vi "externalSetParam.vi"(0 "reference":refnum<class "ClassRelationshipEdge.lvclass">, 1 "arrowHead":T2, 2 "string":string, 3 "node":refnum<class "AbstractNode.lvclass">, 4 "bentStyle":T3, 5 "error in (no error)":errorcluster, 6 "setParam":T4, 7 "ConnectionOffset":cluster{"x":i32, "y":i32}, 9 "lineStyle":T1 caption="stroke") -> (14 "reference out":refnum<class "ClassRelationshipEdge.lvclass">, 19 "error out":errorcluster)   [LabVIEW 2020, in "ClassRelationshipEdge.lvclass"]
doc: "Sets externaly parameters on object"
uses:
  <resource>/Framework/Providers/Open_GDS/UML/ClassRelationshipEdge_class/ClassRelationshipEdge.lvclass
  C:/Program Files (x86)/National Instruments/LabVIEW 2020/resource/Framework/Providers/Open_GDS/UML/SegmentedLineEdge_class/SegmentedLineEdge.lvclass
  C:/Program Files (x86)/National Instruments/LabVIEW 2020/resource/Framework/Providers/Open_GDS/UML/AbstractEdge_class/AbstractEdge.lvclass
  <resource>/Framework/Providers/Open_GDS/UML/ClassRelationshipEdge_class/ExternaSetParamType.ctl
  <resource>/Framework/Providers/Open_GDS/UML/AbstractNode_class/AbstractNode.lvclass
  <resource>/Framework/Providers/Open_GDS/UML/BentStyle_class/BentStyleType.ctl
  <resource>/Framework/Providers/Open_GDS/UML/ArrowHead_class/ArrowHeadType.ctl
  <resource>/Framework/Providers/Open_GDS/UML/LineStyle_class/LineStyleType.ctl
  <resource>/Framework/Providers/Open_GDS/UML/ArrowHead_class/ArrowHead.lvclass
  <resource>/Framework/Providers/Open_GDS/UML/BentStyle_class/BentStyle.lvclass
  <resource>/Framework/Providers/Open_GDS/UML/SegmentedLineEdge_class/SegmentedLineEdge.lvclass
  <resource>/Framework/Providers/Open_GDS/UML/AbstractEdge_class/AbstractEdge.lvclass
  <resource>/Framework/Providers/Open_GDS/UML/LineStyle_class/LineStyle.lvclass
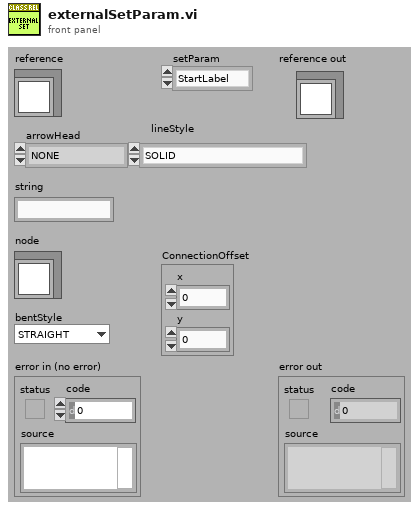
[diagram p1: front panel]
types:
  T1 = typedef "LineStyle.lvclass/LineStyleType.ctl" = enum16{"SOLID", "DOTTED"}
  T2 = typedef "ArrowHead.lvclass/ArrowHeadType.ctl" = enum16{"NONE", "TRIANGLE", "BLACK_TRIANGLE", "V", "HALF_V", "DIAMOND", "BLACK_DIAMOND"}
  T3 = typedef "BentStyle.lvclass/BentStyleType.ctl" = enum16{"STRAIGHT", "HV", "VH", "HVH", "VHV", "ARC"}
  T4 = typedef "ClassRelationshipEdge.lvclass/ExternaSetParamType.ctl" = enum16{"StartLabel", "MidLabel", "EndLabel", "StartNode", "EndNode", "BendType", "StartArrow", "EndArrow", "StartOffset", "EndOffset", "LineStyle"}
  T5 = typedef "ClassRelationshipEdge.lvclass/ObjectAttributes.ctl" = cluster{"bentStyleRef":refnum<class "BentStyle.lvclass">, "startConnectionOffset":cluster{"x":i32, "y":i32}, "endConnectionOffset":cluster{"x":i32, "y":i32}, "MidLineOffset":cluster{"x":i32, "y":i32}, "DepClass":T6}
  T6 = typedef "ReversedEngineering_ViDependencyDetailsType.ctl" = cluster{"ThisVIs/Ctls":path[], "Dependent_VIs/Ctls":path[]}
  T7 = typedef "SegmentedLineEdge.lvclass/ObjectAttributes.ctl" = cluster{"lineStyle":refnum<class "LineStyle.lvclass">, "startArrowHead":refnum<class "ArrowHead.lvclass">, "endArrowHead":refnum<class "ArrowHead.lvclass">, "startLabel":string, "midLabel":string, "endLabel":string, "MidLabelOffset":T8, "SplitWire":bool}
  T8 = typedef "Point Point2D.ctl" = cluster{"x":dbl, "y":dbl}
  T9 = typedef "AbstractEdge.lvclass/ObjectAttributes.ctl" = cluster{"start":refnum<class "AbstractNode.lvclass">, "end":refnum<class "AbstractNode.lvclass">}
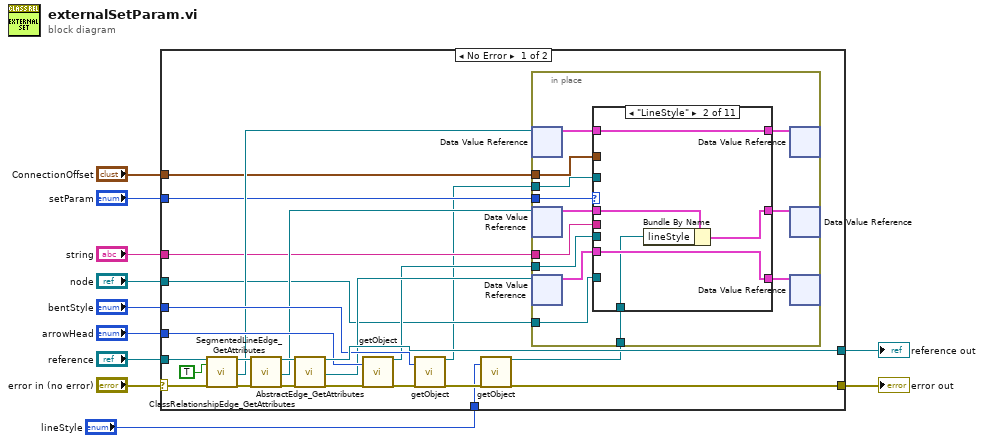
[diagram p0: block diagram]
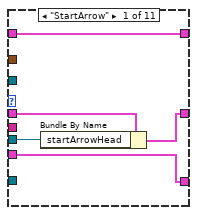
[diagram p2: hidden frame]
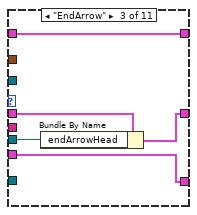
[diagram p3: hidden frame]
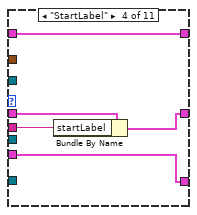
[diagram p4: hidden frame]
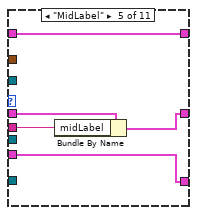
[diagram p5: hidden frame]
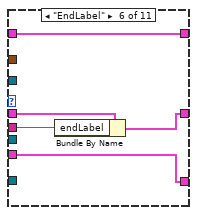
[diagram p6: hidden frame]
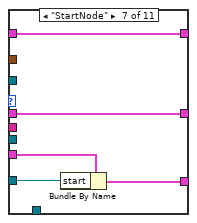
[diagram p7: hidden frame]
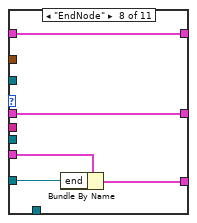
[diagram p8: hidden frame]
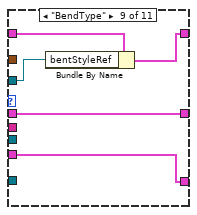
[diagram p9: hidden frame]
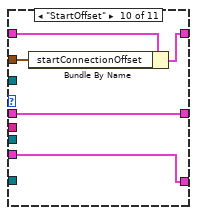
[diagram p10: hidden frame]
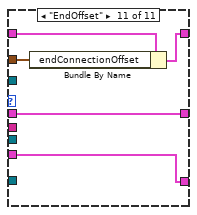
[diagram p11: hidden frame]
diagram:
  n1 = case shown="No Error" "error in (no error)" {
    selector: "error in (no error)" -> [w36 w105]
    tunnel: "reference" -> [w35 w106]
    tunnel: [w14 w105] -> w9
    tunnel: [w34 w106] -> w8
    tunnel: "setParam" -> [w21 _]
    tunnel: "string" -> [w20 _]
    tunnel: "arrowHead" -> [w33 _]
    tunnel: "node" -> [w18 _]
    tunnel: "bentStyle" -> [w32 _]
    tunnel: "ConnectionOffset" -> [w16 _]
    tunnel: "lineStyle" -> [w12 _]
    frame No Error {
      n2 = call <resource>:"ClassRelationshipEdge_GetAttributes.vi"("reference in"=w35, "OnlyGetDvrReference(False)"=TRUE, "error in (no error)"=w36) -> ("reference out"=w29:refnum<class "ClassRelationshipEdge.lvclass">, "DataRef"=w24:refnum<data-value>, "error out"=w28:errorcluster)  [unwired: 13 in, 1 out]
      n3 = call <resource>:"SegmentedLineEdge_GetAttributes.vi"("reference in"=w29, "error in (no error)"=w28) -> ("reference out"=w27:refnum<class "ClassRelationshipEdge.lvclass">, "DataRef"=w23:refnum<data-value>, "error out"=w26:errorcluster)  [unwired: 14 in, 1 out]
      n4 = call <resource>:"AbstractEdge_GetAttributes.vi"("reference in"=w27, "error in (no error)"=w26) -> ("reference out"=w34:refnum<class "ClassRelationshipEdge.lvclass">, "DataRef"=w22:refnum<data-value>, "error out"=w25:errorcluster)  [unwired: 14 in, 1 out]
      n5 = call <resource>:"getObject.vi"("arrowHead"=w33, "error in (no error)"=w25) -> ("reference out"=w19:refnum<class "ArrowHead.lvclass">, "error out"=w31:errorcluster)  [unwired: 16 out]
      n6 = call <resource>:"getObject.vi"("bentStyle"=w32, "error in (no error)"=w31) -> ("reference out"=w17:refnum<class "BentStyle.lvclass">, "error out"=w15:errorcluster)  [unwired: 16 out]
      n7 = call <resource>:"getObject.vi"("lineStyle"=w12, "error in (no error)"=w15) -> ("reference out"=w13:refnum<class "LineStyle.lvclass">, "error out"=w14:errorcluster)  [unwired: 16 in]
      n8 = in-place {
        in-place-border: w21 -> [w49]
        in-place-border: w20 -> [w48]
        in-place-border: w19 -> [w47]
        in-place-border: w18 -> [w46]
        in-place-border: w17 -> [w45]
        in-place-border: w16 -> [w38]
        in-place-border: w13 -> [w37]
        n9 = in-place-dvr #1(w24) -> (w42:T5)  [unwired: 1 out]
        n10 = in-place-dvr #2(w23) -> (w44:T7)  [unwired: 1 out]
        n11 = in-place-dvr #3(w22) -> (w43:T9)  [unwired: 1 out]
        n12 = case shown="\"LineStyle\"" w49 {
          tunnel: [w54 w59 w62 w69 w74 w79 w81 w85 w90 w96 w101] -> w41
          tunnel: w48 -> [_ _ _ w68 w73 w78 _ _ _ _ _]
          tunnel: w47 -> [w53 _ w64 _ _ _ _ _ _ _ _]
          tunnel: w46 -> [_ _ _ _ _ _ w84 w89 _ _ _]
          tunnel: w45 -> [_ _ _ _ _ _ _ _ w94 _ _]
          tunnel: w44 -> [w52 w58 w63 w67 w72 w77 w81 w85 w90 w96 w101]
          tunnel: w43 -> [w51 w57 w61 w66 w71 w76 w83 w88 w91 w97 w102]
          tunnel: w42 -> [w50 w56 w60 w65 w70 w75 w80 w86 w93 w99 w104]
          tunnel: [w51 w57 w61 w66 w71 w76 w82 w87 w91 w97 w102] -> w40
          tunnel: [w50 w56 w60 w65 w70 w75 w80 w86 w92 w98 w103] -> w39
          tunnel: w38 -> [_ _ _ _ _ _ _ _ _ w95 w100]
          tunnel: w37 -> [_ w55 _ _ _ _ _ _ _ _ _]
          frame "StartArrow" {
            n13 = Bundle By Name(cluster=w52, "startArrowHead"=w53) -> (w54:T7)
          }
          frame "LineStyle" {
            n14 = Bundle By Name(cluster=w58, "lineStyle"=w55) -> (w59:T7)
          }
          frame "EndArrow" {
            n15 = Bundle By Name(cluster=w63, "endArrowHead"=w64) -> (w62:T7)
          }
          frame "StartLabel" {
            n16 = Bundle By Name(cluster=w67, "startLabel"=w68) -> (w69:T7)
          }
          frame "MidLabel" {
            n17 = Bundle By Name(cluster=w72, "midLabel"=w73) -> (w74:T7)
          }
          frame "EndLabel" {
            n18 = Bundle By Name(cluster=w77, "endLabel"=w78) -> (w79:T7)
          }
          frame "StartNode" {
            n19 = Bundle By Name(cluster=w83, "start"=w84) -> (w82:T9)
          }
          frame "EndNode" {
            n20 = Bundle By Name(cluster=w88, "end"=w89) -> (w87:T9)
          }
          frame "BendType" {
            n21 = Bundle By Name(cluster=w93, "bentStyleRef"=w94) -> (w92:T5)
          }
          frame "StartOffset" {
            n22 = Bundle By Name(cluster=w99, "startConnectionOffset"=w95) -> (w98:T5)
          }
          frame "EndOffset" {
            n23 = Bundle By Name(cluster=w104, "endConnectionOffset"=w100) -> (w103:T5)
          }
        }
        n24 = in-place-dvr #1(w39) -> ()  [unwired: 2 out]
        n25 = in-place-dvr #2(w41) -> ()  [unwired: 2 out]
        n26 = in-place-dvr #3(w40) -> ()  [unwired: 2 out]
      }
    }
    frame Error {
    }
  }
  "reference out" <- w8
  "error out" <- w9
